vi "StopQ0Stream.vi"(8 "error in (no error)":errorcluster, 11 "Scope5761 in":refnum<class "Scope5782_six_channel.lvclass">) -> (0 "error out":errorcluster, 3 "Scope5761 out":refnum<class "Scope5782_six_channel.lvclass">)   [LabVIEW 2025, in "Scope5782_six_channel.lvclass"]
uses:
  Scope5782_six_channel.lvclass
  FileStream/DumpFileAction.ctl
  Scope5782_six_channel.lvclass/Scope5782_six_channel.ctl
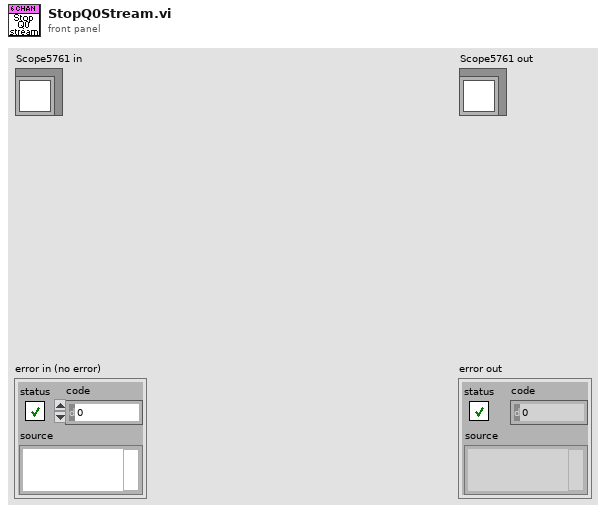
[diagram p1: front panel]
types:
  T1 = typedef "DumpFileAction.ctl" = enum16{"StartNew", "StartAppend", "Data", "Close"}
  T2 = typedef "DumpFileQueue.ctl" = refnum<queue>
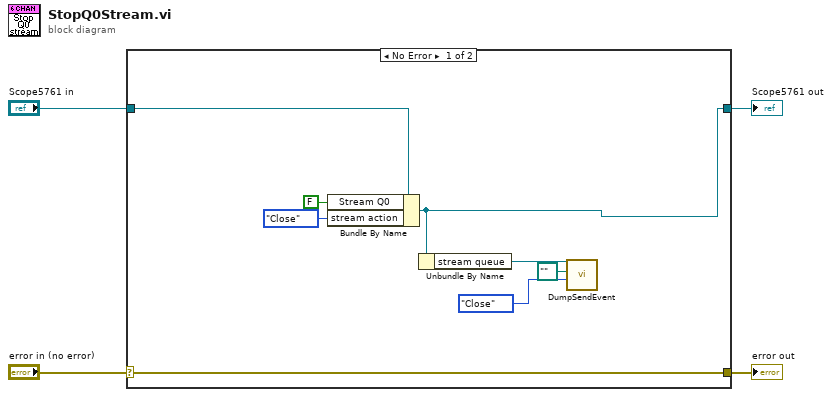
[diagram p0: block diagram]
diagram:
  n1 = case shown="No Error" "error in (no error)" {
    selector: "error in (no error)" -> [w12 w14]
    tunnel: [w12 w14] -> w3
    tunnel: [w8 w13] -> w1
    tunnel: "Scope5761 in" -> [w10 w13]
    frame No Error {
      n2 = Bundle By Name(cluster=w10, "Stream Q0"=FALSE, "stream action"=DumpFileAction."Close") -> (w8:refnum<class "Scope5782_six_channel.lvclass">)
      n3 = Unbundle By Name(w8) -> ("stream queue"=w7:T2)
      n4 = call "DumpSendEvent.vi"("DumpFileAction"=DumpFileAction."Close", "Path"=path "", "DumpFileQueue"=w7) -> ()  [unwired: 9 in]
    }
    frame Error {
    }
  }
  "error out" <- w3
  "Scope5761 out" <- w1
